vi "TrajectoryGenerate_Make_Cubic.vi"(8 "traj_config":T6 {"End Velocity" format="%20.4f"; "StartVelocity" format="%20.4f"; "Max Acceleration" format="%20.4f"; "MaxVelocity" format="%20.4f"}, 9 "Enging POSE":T3={"TRANSLATION"={"X"=0.0, "Y"=0.0}, "ROTATION"={"VALUE"=0.0, "COS"=1.0, "SIN"=0.0}} {"ROTATION"."SIN" format="%13.4f"; "ROTATION"."COS" format="%13.4f"; "ROTATION"."VALUE" format="%13.4f"; "TRANSLATION"."Y" format="%14.3f"; "TRANSLATION"."X" format="%14.3f"}, 10 "Interior WAYPOINTS":T4[](array[typedef]) {"Y" format="%14.3f"; "X" format="%14.3f"}, 11 "Starting POSE":T3={"TRANSLATION"={"X"=0.0, "Y"=0.0}, "ROTATION"={"VALUE"=0.0, "COS"=1.0, "SIN"=0.0}} {"ROTATION"."SIN" format="%13.4f"; "ROTATION"."COS" format="%13.4f"; "ROTATION"."VALUE" format="%13.4f"; "TRANSLATION"."Y" format="%14.3f"; "TRANSLATION"."X" format="%14.3f"}) -> (0 "error out":errorcluster, 3 "TRAJECTORY":T1 {"States"."POSE"."ROTATION"."SIN" format="%13.4f"; "States"."POSE"."ROTATION"."COS" format="%13.4f"; "States"."POSE"."ROTATION"."VALUE" format="%13.4f"; "States"."POSE"."TRANSLATION"."Y" format="%14.3f"; "States"."POSE"."TRANSLATION"."X" format="%14.3f"; "TotalTImeSecs" format="%20.3f"})   [LabVIEW 2019, in "Trajectory_Library.lvlib"]
doc: "Generates a trajectory from the given waypoints and config. This method uses clamped cubic splines -- a method in which the initial pose, final pose, and interior waypoints are provided. The headings are automatically determined at the interior points to ensure continuous curvature. \nParameters:\n - startingPose - The initial Pose.\n - interiorWaypoints - The interior waypoints.\n - ending Pose - The ending Pose.\n - Trajectory Config - The configuration for the trajectory.\n\nReturns:\n - Trajectory -- Created trajectory data structure\n - Error Out - Returned error cluster"
uses:
  Trajectory_Library.lvlib
  TypeDef/TRANSLATION2D.ctl
  TypeDef/ROTATION2D.ctl
  TypeDef/POSE2D.ctl
  TypeDef/TRAJ_CONFIG.ctl
  TypeDef/TRAJ_STATE.ctl
  TypeDef/TRAJECTORY.ctl
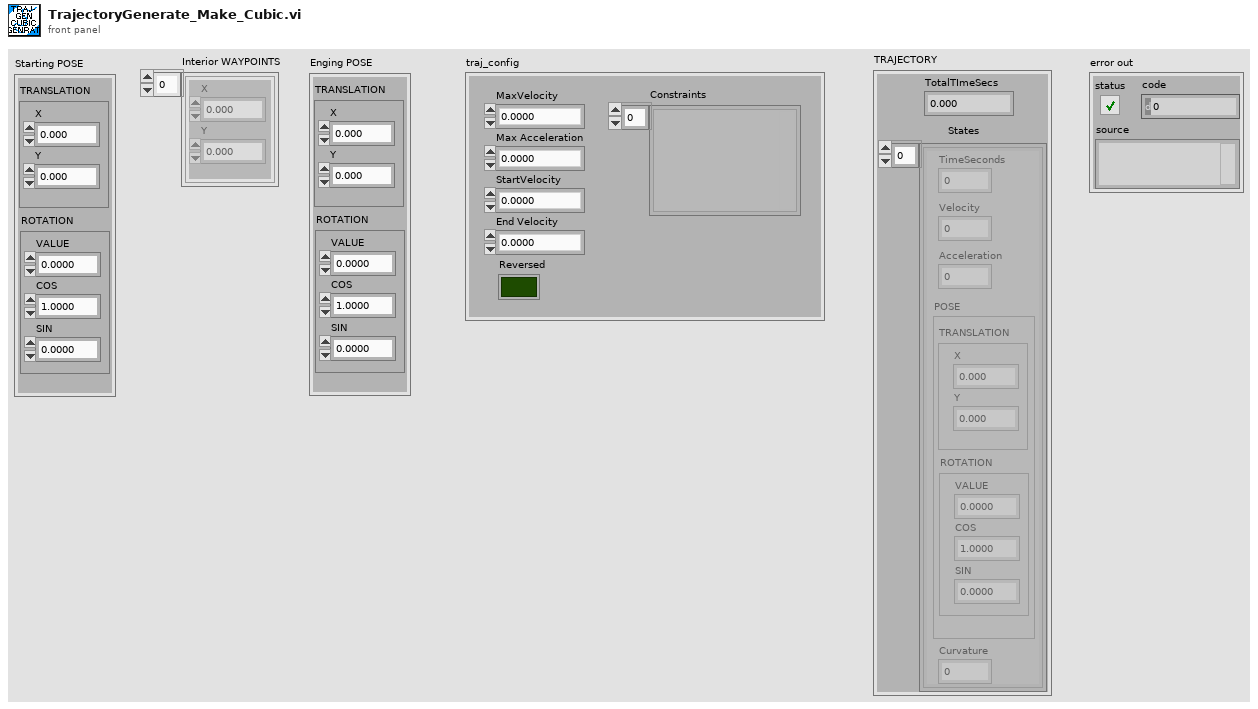
[diagram p1: front panel]
types:
  T1 = typedef "Trajectory_Library.lvlib/TRAJECTORY.ctl" = cluster{"TotalTImeSecs":dbl, "States":T2[]}
  T2 = typedef "Trajectory_Library.lvlib/TRAJ_STATE.ctl" = cluster{"TimeSeconds":dbl, "Velocity":dbl, "Acceleration":dbl, "POSE":T3, "Curvature":dbl}
  T3 = typedef "Trajectory_Library.lvlib/POSE2D.ctl" = cluster{"TRANSLATION":T4, "ROTATION":T5}
  T4 = typedef "Trajectory_Library.lvlib/TRANSLATION2D.ctl" = cluster{"X":dbl, "Y":dbl}
  T5 = typedef "Trajectory_Library.lvlib/ROTATION2D.ctl" = cluster{"VALUE":dbl, "COS":dbl, "SIN":dbl}
  T6 = typedef "Trajectory_Library.lvlib/TRAJ_CONFIG.ctl" = cluster{"MaxVelocity":dbl, "Max Acceleration":dbl, "StartVelocity":dbl, "End Velocity":dbl, "Reversed":bool, "Constraints":variant[]}
  T7 = typedef "WPILib_Math.lvlib/SPLINE_CTRL_VECTOR.ctl" = cluster{"Xs":dbl[], "Ys":dbl[]}
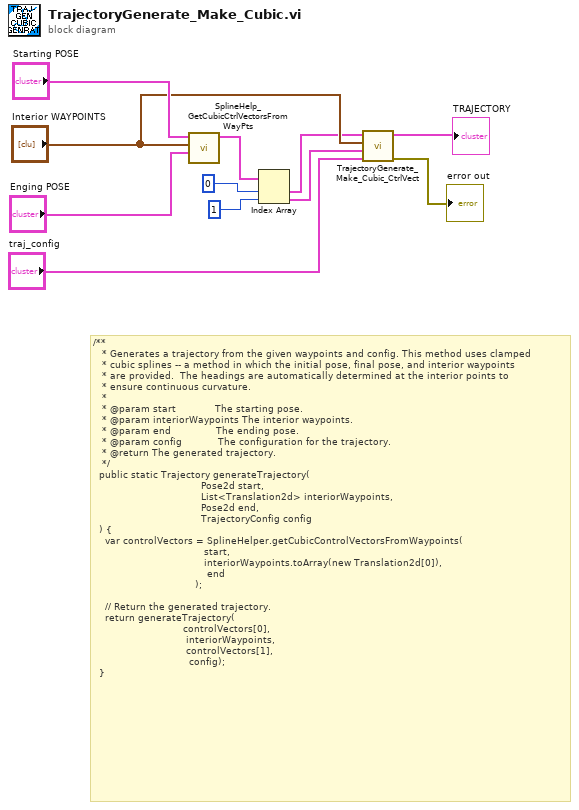
[diagram p0: block diagram]
diagram:
  # "/**\n   * Generates a trajectory from the given waypoints and config. This method uses clamped\n   * cubic splines -- a method in which the initial pose, final pose, and interior waypoints\n   * are provided.  The headings are automatically determined at the interior points to\n   * ensure continuous curvature.\n   *\n   * @param start             The starting pose.\n   * @param interiorWaypoints The interior waypoints.\n   * @param end               The ending pose.\n   * @param config            The configuration for the trajectory.\n   * @return The generated trajectory.\n   */\n  public static Trajectory generateTrajectory(\n                                    Pose2d start, \n                                    List<Translation2d> interiorWaypoints, \n                                    Pose2d end,\n                                    TrajectoryConfig config\n  ) {\n    var controlVectors = SplineHelper.getCubicControlVectorsFromWaypoints(\n                                     start, \n                                     interiorWaypoints.toArray(new Translation2d[0]), \n                                      end\n                                  );\n\n    // Return the generated trajectory.\n    return generateTrajectory(   \n                              controlVectors[0], \n                               interiorWaypoints, \n                               controlVectors[1], \n                                config);\n  }"
  n1 = call "SplineHelp_GetCubicCtrlVectorsFromWayPts.vi"("Enging POSE"="Enging POSE", "Interior WAYPOINTS"="Interior WAYPOINTS", "Starting POSE"="Starting POSE") -> ("SplineControlVectors"=w4:T7[])  [unwired: 8 in]
  n2 = Index Array(array=w4, index #1=0 ("index"), index #2=1 ("index")) -> (element #1=w3:T7, element #2=w2:T7)
  n3 = call "TrajectoryGenerate_Make_Cubic_CtrlVect.vi"("traj_config"="traj_config", "end-Spline_Ctrl_Vector"=w2, "Interior WAYPOINTS"="Interior WAYPOINTS", "initial-Spline_Ctrl_Vector"=w3) -> ("error out"=→"error out":errorcluster, "TRAJECTORY"=→"TRAJECTORY":T1)  [unwired: 6 in]
